vi "Virtual DAQ Messauftrag einstellen.vi"(0 "Messart":T2(ring), 1 "Physikalischer Kanal":string, 2 "PFI Klemme":string, 3 "Abtastrate Hz":dbl=1000.0, 4 "Samples pro Block":i32=100, 5 "Spannungsbereich ±V":dbl=10.0, 6 "Kontinuierlich":bool) -> (20 "Auftrag":T1={"Messart"=enum."Wahl treffen", "Kanal"="", "PFI"="", "Rate"=1000.0, "Samples"=100, "Bereich"=10.0, "Kontinuierlich"=FALSE})   [LabVIEW 2026]
doc: "Erstellt den Typ fuer PuT3 DAQ.vi. Hier Messart, Kanal, Bereich und Abtastung einstellen. Die Steckwerkbank wird erst beim Aufruf von PuT3 DAQ angesprochen."
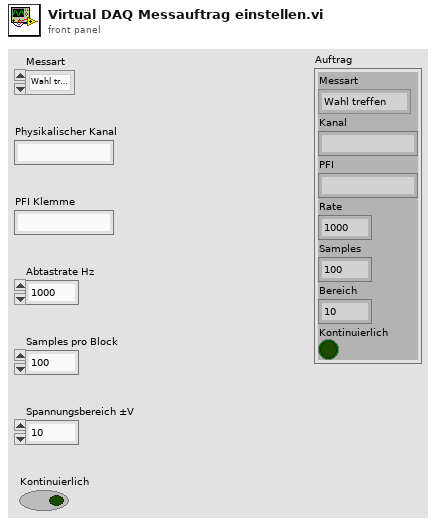
[diagram p1: front panel]
types:
  T1 = cluster{"Messart":enum8{"Wahl treffen", "AI Spannung", "AO Spannung", "DI Lesen", "DO Schreiben", "CTR Frequenz", "DMM Widerstand", "Ausgaenge freigeben"}, "Kanal":string, "PFI":string, "Rate":dbl, "Samples":i32, "Bereich":dbl, "Kontinuierlich":bool}
  T2 = enum8{"Wahl treffen", "AI Spannung", "AO Spannung", "DI Lesen", "DO Schreiben", "CTR Frequenz", "DMM Widerstand", "Ausgaenge freigeben"}
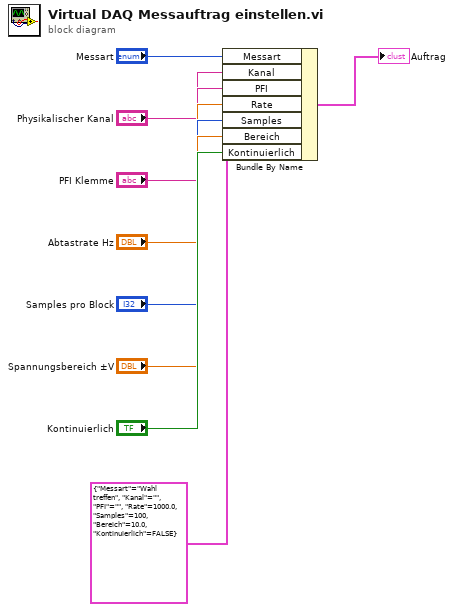
[diagram p0: block diagram]
diagram:
  n1 = Bundle By Name(cluster=T1 {"Messart"=enum."Wahl treffen", "Kanal"="", "PFI"="", "Rate"=1000.0, "Samples"=100, "Bereich"=10.0, "Kontinuierlich"=FALSE}, "Messart"="Messart", "Kanal"="Physikalischer Kanal", "PFI"="PFI Klemme", "Rate"="Abtastrate Hz", "Samples"="Samples pro Block", "Bereich"="Spannungsbereich ±V", "Kontinuierlich"="Kontinuierlich") -> (→"Auftrag":T1)
